vi "Is Software Trigger Supported.vi"(8 "error in (no error)":errorcluster, 11 "Camera in":refnum<class "Camera.lvclass">) -> (0 "error out":errorcluster, 2 "Supported":bool, 3 "Camera":refnum<class "Camera.lvclass">)   [LabVIEW 2020, in "Camera.lvclass"]
uses:
  Camera.lvclass
  Camera.lvclass/Camera.ctl
  bin/gindustrialcam_32-1.dll
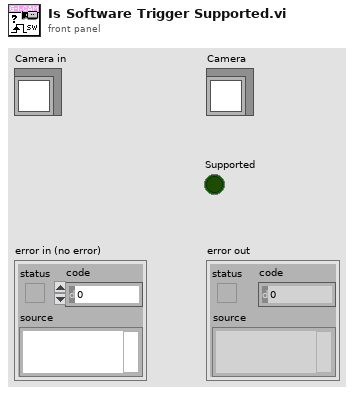
[diagram p1: front panel]
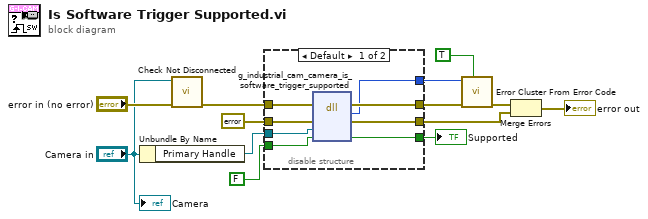
[diagram p0: block diagram]
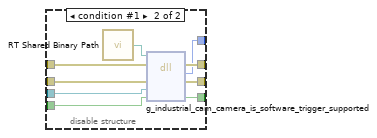
[diagram p2: hidden frame]
diagram:
  n1 = Unbundle By Name("Camera in") -> ("Primary Handle"=w5:refnum<data-value>)
  n2 = call "Check Not Disconnected.vi"("error in (no error)"="error in (no error)", "Camera in"="Camera in") -> ("error out"=w4:errorcluster)  [unwired: 9 in]
  n3 = disable-structure shown="Default" {
    disable-tunnel: [w21 w30] -> w11
    disable-tunnel: [w20 w29] -> w10
    disable-tunnel: [w19 w28] -> w8
    disable-tunnel: errorcluster {"status"=FALSE, "code"=0, "source"=""} ("error constant") -> [w18 w27]
    disable-tunnel: w5 -> [w17 w26]
    disable-tunnel: w4 -> [w16 w25]
    disable-tunnel: FALSE -> [w15 w24]
    disable-tunnel: [w14 w23] -> w1
    frame condition #0 (active) {
      n4 = dll-call lib="C:/serenial/lib/g-industrial-camera/LabVIEW/g_industrial_cam/bin/gindustrialcam_*-1.*" fn="g_industrial_cam_camera_is_software_trigger_supported"(error in=w16, "err"=w18, "edvr"=w17, "supported"=w15) -> (error out=w21:errorcluster, "Mg_Error"=w20:i32, "err"=w19:errorcluster, "supported"=w14:bool)  [unwired: 3 in, 1 out]
    }
    frame condition #1 {
      n5 = call "RT Shared Binary Path.vi"() -> ("Path"=w22:path)
      n6 = dll-call lib="C:/serenial/lib/g-industrial-camera/LabVIEW/g_industrial_cam/bin/gindustrialcam_*-1.*" fn="g_industrial_cam_camera_is_software_trigger_supported"(path in=w22, error in=w25, "err"=w27, "edvr"=w26, "supported"=w24) -> (error out=w30:errorcluster, "Mg_Error"=w29:i32, "err"=w28:errorcluster, "supported"=w23:bool)  [unwired: 2 in, 1 out]
    }
  }
  "Supported" <- w1
  n7 = call <vilib>:"Error Cluster From Error Code.vi"("show call chain? (False)"=TRUE, "error in (no error)"=w11, "error code (0)"=w10) -> ("error out"=w9:errorcluster)  [unwired: 6 in]
  n8 = Merge Errors(w9, w8) -> (→"error out":errorcluster)
  "Camera" <- "Camera in"
